vi "convert_current_to_power.vi"(9 "Measured Power Refnum":refnum<vi>, 10 "Current Ref":refnum<vi>, 11 "Power Threshold":cluster{"Value":dbl, "Units":dbl}={"Value"=0.5, "Units"=0.001} {"Units" items=["mW"=0.001, "W"=1.0]; "Value" min=0.0 step=50.0}) -> (2 "Power Out":cluster{"Value":dbl, "Units":dbl}={"Value"=0.0, "Units"=0.001} {"Units" items=["mW"=0.001, "W"=1.0]; "Value" min=0.0 step=50.0}, 3 "Current Out":cluster{"Value":dbl, "Units":dbl}={"Value"=0.0, "Units"=0.001} {"Units" items=["mA"=0.001, "A"=1.0]; "Value" min=0.0 step=50.0})   [LabVIEW 2025, in "tSNIP.lvlib"]
uses:
  tSNIP.lvlib
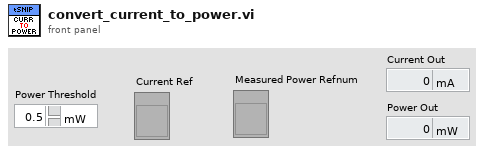
[diagram p1: front panel]
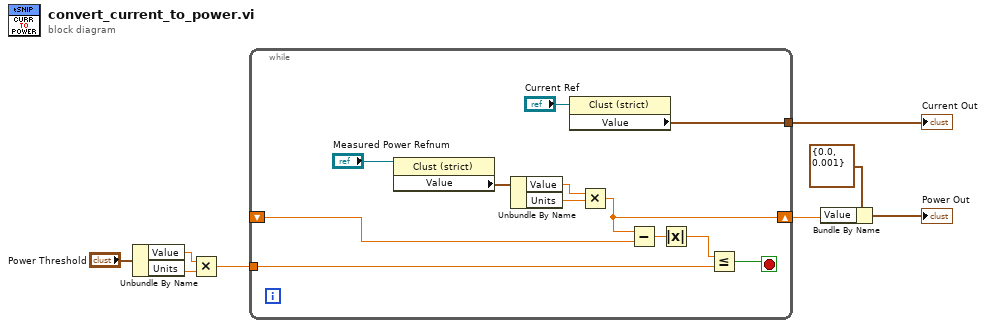
[diagram p0: block diagram]
diagram:
  n1 = Unbundle By Name("Power Threshold") -> ("Value"=w7:dbl, "Units"=w6:dbl)
  n2 = Multiply(x=w7, y=w6) -> (x*y=w5:dbl)
  n3 = while {
    shift-right: [w9] -> w4
    shift-left: _ -> [w19]
    tunnel: w5 -> [w16]
    tunnel: [w13] -> w1
    stop <- w15 stop-if-true
    n4 = property class="Clust (strict)"(reference="Measured Power Refnum") -> ("Value"=w12:cluster{"Value":dbl, "Units":dbl})  [unwired: 1 in, 2 out]
    n5 = Unbundle By Name(w12) -> ("Value"=w10:dbl, "Units"=w11:dbl)
    n6 = property class="Clust (strict)"(reference="Current Ref") -> ("Value"=w13:cluster{"Value":dbl, "Units":dbl})  [unwired: 1 in, 2 out]
    n7 = Multiply(x=w10, y=w11) -> (x*y=w9:dbl)
    n8 = Subtract(x=w9, y=w19) -> (x-y=w18:dbl)
    n9 = Absolute Value(x=w18) -> (abs(x)=w17:dbl)
    n10 = Less Or Equal?(x=w17, y=w16) -> (x <= y?=w15:bool)
  }
  "Current Out" <- w1
  n11 = Bundle By Name(cluster=cluster{"Value":dbl, "Units":dbl} {"Value"=0.0, "Units"=0.001} ("Steady State Power"), "Value"=w4) -> (→"Power Out":cluster{"Value":dbl, "Units":dbl})
